vi "test.vi"(8 "error in (no error)":errorcluster, 11 "YoutuberDownloader":refnum<class "YoutuberDownloader.lvclass">) -> (0 "error out":errorcluster, 3 "estimatedTime":u32)   [LabVIEW 2018, in "Demo.lvclass"]
uses:
  Demo.lvclass
  YoutuberDownloader Class/YoutuberDownloader.lvclass
  ConsoleOut/Print Options.ctl
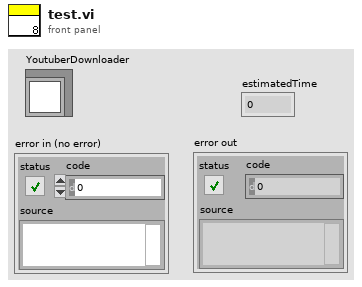
[diagram p1: front panel]
types:
  T1 = typedef "Print Options.ctl" = enum16{"Create", "Get Reference", "Print", "Print Header", "Close"}
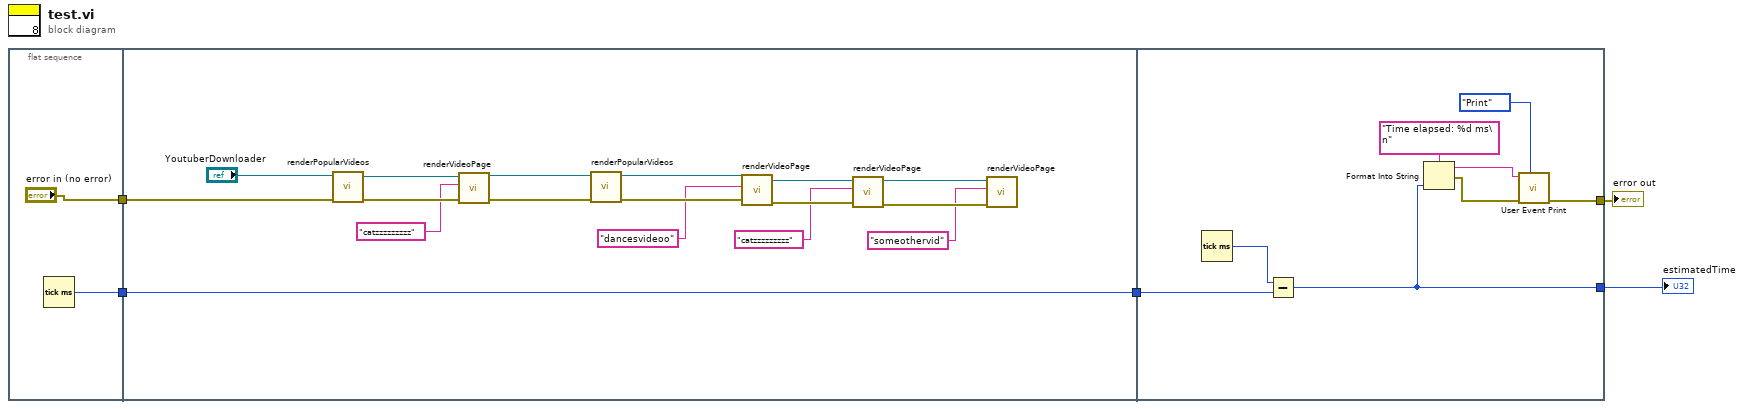
[diagram p0: block diagram]
diagram:
  n1 = flat-sequence {
    tunnel: [w7] -> w5
    tunnel: ["error in (no error)"] -> w1
    tunnel: w5 -> [w9]
    tunnel: [w9] -> w4
    tunnel: w1 -> [w8]
    tunnel: w4 -> [w31]
    tunnel: [w29] -> w3
    tunnel: [w25] -> w2
    frame #0 {
      n2 = Tick Count (ms)() -> (millisecond timer value=w7:u32)
    }
    frame #1 {
      n3 = call "renderPopularVideos.vi"("error in (no error)"=w8, "YoutuberDownloader in"="YoutuberDownloader") -> ("error out"=w22:errorcluster, "YoutuberDownloader out"=w23:refnum<class "YoutuberDownloader.lvclass">)  [unwired: 8 in]
      n4 = call "renderVideoPage.vi"("error in (no error)"=w22, "VideoId"="catzzzzzzzzz", "YoutuberDownloader in"=w23) -> ("error out"=w19:errorcluster, "YoutuberDownloader out"=w20:refnum<class "YoutuberDownloader.lvclass">)  [unwired: 7 in]
      n5 = call "renderPopularVideos.vi"("error in (no error)"=w19, "YoutuberDownloader in"=w20) -> ("error out"=w17:errorcluster, "YoutuberDownloader out"=w18:refnum<class "YoutuberDownloader.lvclass">)  [unwired: 8 in]
      n6 = call "renderVideoPage.vi"("error in (no error)"=w17, "VideoId"="dancesvideoo", "YoutuberDownloader in"=w18) -> ("error out"=w12:errorcluster, "YoutuberDownloader out"=w13:refnum<class "YoutuberDownloader.lvclass">)  [unwired: 7 in]
      n7 = call "renderVideoPage.vi"("error in (no error)"=w12, "VideoId"="catzzzzzzzzz", "YoutuberDownloader in"=w13) -> ("error out"=w14:errorcluster, "YoutuberDownloader out"=w15:refnum<class "YoutuberDownloader.lvclass">)  [unwired: 7 in]
      n8 = call "renderVideoPage.vi"("error in (no error)"=w14, "VideoId"="someothervid", "YoutuberDownloader in"=w15) -> ()  [unwired: 7 in, 2 out]
    }
    frame #2 {
      n9 = Tick Count (ms)() -> (millisecond timer value=w32:u32)
      n10 = Subtract(x=w32, y=w31) -> (x-y=w29:u32)
      n11 = Format Into String(format string="Time elapsed: %d ms\n", w29) -> (resulting string=w28:string, error out=w27:errorcluster)  [unwired: 2 in]
      n12 = call "User Event Print.vi"("Options"=Print_Options."Print", "error in (no error)"=w27, "String to Print"=w28) -> ("error out"=w25:errorcluster)  [unwired: 7 in, 1 out]
    }
  }
  "estimatedTime" <- w3
  "error out" <- w2
